vi "CSE ISP - path of example scripts.vi"(7 "subdir":string="Example Scripts", 8 "error in":errorcluster, 9 "pattern":string="*.ces", 10 "file":string) -> (0 "error out":errorcluster, 1 "extension":string, 2 "file path":path, 3 "path of example scripts":path, 4 "pattern out":string)   [LabVIEW 2021]
doc: "::: CalcExpress Toolkit :::\nCopyright (c) 2000-2026 Konstantin Shifershteyn. All rights reserved."
uses:
  vi.lib/addons/CalcExpress/cemisc.llb/[ce] CE component paths - Kind of Path Enum.ctl
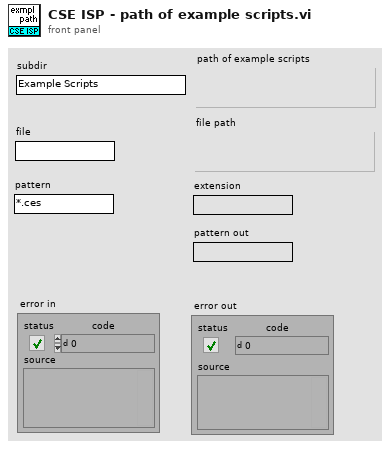
[diagram p1: front panel]
types:
  T1 = typedef "[ce] CE component paths - Kind of Path Enum.ctl" = enum16{"VIs", "FuncVIs", "Help", "Examples", "Project", "Templates"}
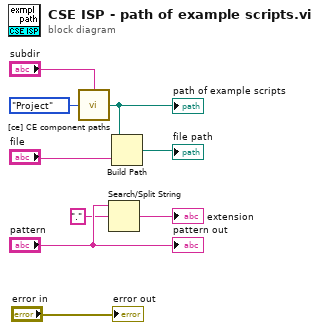
[diagram p0: block diagram]
diagram:
  n1 = call "[ce] CE component paths.vi"("kind of path"=[ce]_CE_component_paths_-_Kind_of_Path_Enum."Project", "append path"="subdir") -> ("path out"=w4:path)
  "path of example scripts" <- w4
  n2 = Search/Split String(string="pattern", search string/char (-)="." ("search char (-)")) -> (match + rest of string=→"extension":string)  [unwired: 1 in, 2 out]
  n3 = Build Path(base path=w4, name or relative path="file") -> (appended path=→"file path":path)
  "pattern out" <- "pattern"
  "error out" <- "error in"
